vi "Draw Shapes.vi"(0 "Picture in":refnum<vi>, 1 "Commands":cluster{"Time (s)":dbl, T1, "Enabled":bool}[](array[cluster]), 3 "Sample Period (s)":dbl=0.02, 5 "Points":cluster{"x":dbl, "y":dbl, "th":dbl}[](array[cluster]), 7 "Valid Path?":bool=TRUE, 9 "new picture in":picture, 11 "Results":T4, 13 "Output Point":T3, 14 "Path Points":cluster{"x":dbl, "y":dbl}[](array[cluster])) -> (4 "new picture out":picture)   [LabVIEW 2023]
uses:
  Types/Single Cmd Info.ctl
  <vilib>/picture/picture.llb/imagedata.ctl
  Global Settings.vi
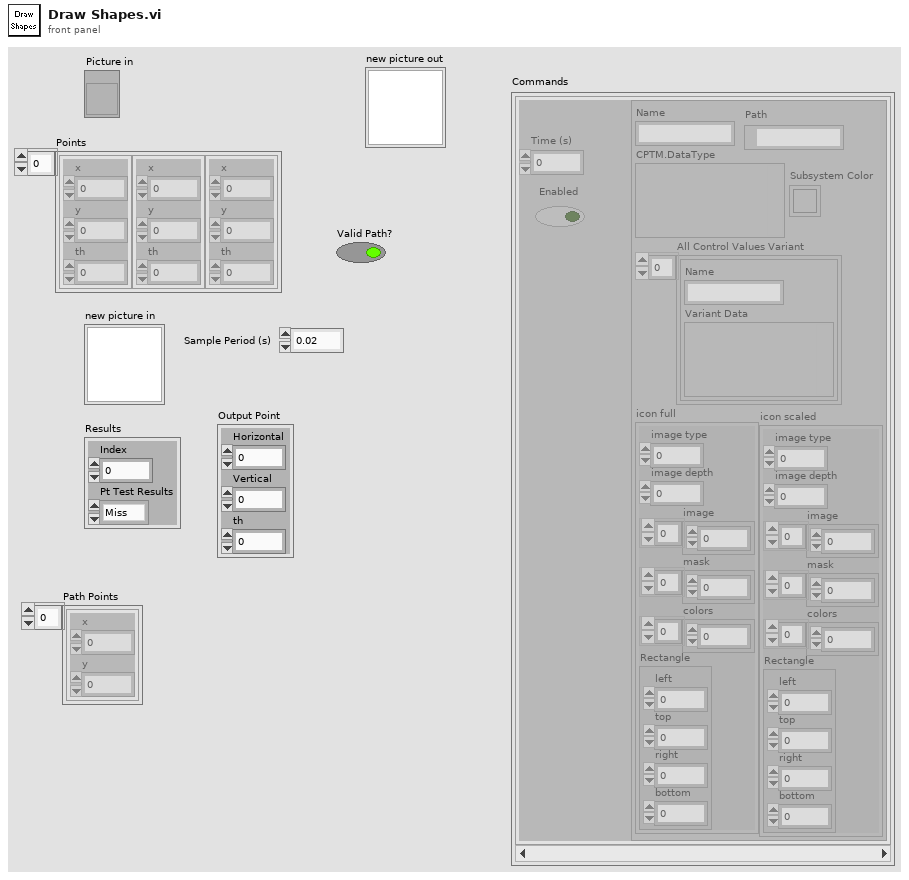
[diagram p1: front panel]
types:
  T1 = typedef "Single Cmd Info.ctl" = cluster{"Name":string, "CPTM.DataType":variant, "All Control Values Variant":cluster{"Name":string, "Variant Data":variant}[], "icon full":T2, "icon scaled":T2, "Path":path, "Subsystem Color":u32}
  T2 = typedef "imagedata.ctl" = cluster{"image type":i32, "image depth":i32, "image":u8[], "mask":u8[], "colors":u32[], "Rectangle":cluster{"left":i16, "top":i16, "right":i16, "bottom":i16}}
  T3 = cluster{"Horizontal":dbl, "Vertical":dbl, "th":dbl}
  T4 = cluster{"Index":i32, "Pt Test Results":enum16{"Miss", "Rect Hit", "Arrow Hit"}}
  T5 = typedef "LVPositionTypeDef.ctl" = cluster{"Left":i32, "Top":i32}
  T6 = typedef "LVBoundsTypeDef.ctl" = cluster{"Width":u32, "Height":u32}
  T7 = cluster{"left":i16, "top":i16, "right":i16, "bottom":i16}
  T8 = cluster{"Horizontal":dbl, "Vertical":dbl, "Horizontal":dbl, "Vertical":dbl}
  T9 = cluster{i32, "Pt Test Results":enum16{"Miss", "Rect Hit", "Arrow Hit"}}
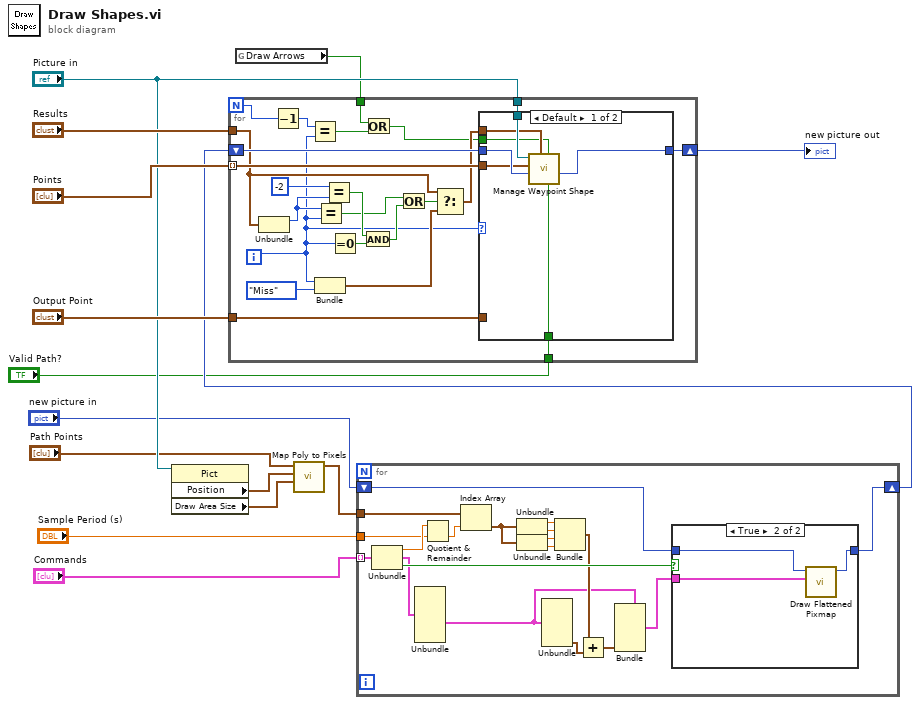
[diagram p0: block diagram]
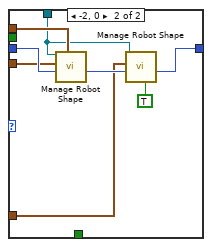
[diagram p3: hidden frame]
diagram:
  n1 = property on="Property Node" class="Pict"(reference="Picture in") -> ("Position"=w9:T5, "Draw Area Size"=w10:T6)  [unwired: 1 in, 2 out]
  n2 = global read "Global Settings.vi" "Draw Arrows"() -> (w2:bool)
  n3 = call "Map Poly to Pixels.vi"("Draw Area Size"=w10, "Position"=w9, "Coords"="Path Points") -> ("Coords"=w7:cluster{"Horizontal":dbl, "Vertical":dbl}[])  [unwired: 8 in]
  n4 = for {
    shift-right: [w27] -> w4
    shift-left: "new picture in" -> [w29]
    tunnel: "Commands" -> [w34] mode=indexing
    tunnel: w7 -> [w33]
    tunnel: "Sample Period (s)" -> [w31]
    n5 = Unbundle(w34) -> ("Time (s)"=w32:dbl, w25:T1, "Enabled"=w28:bool)
    n6 = Unbundle(w25) -> ("icon scaled"=w17:T2)  [unwired: 6 out]
    n7 = Quotient & Remainder(x=w32, y=w31) -> (floor(x/y)=w30:dbl)  [unwired: 1 out]
    n8 = Index Array(array=w33, index=w30) -> (element=w16:cluster{"Horizontal":dbl, "Vertical":dbl})
    n9 = Unbundle(w16) -> ("Horizontal"=w24:dbl, "Vertical"=w23:dbl)
    n10 = Unbundle(w16) -> ("Horizontal"=w22:dbl, "Vertical"=w21:dbl)
    n11 = Unbundle(w17) -> ("Rectangle"=w19:T7)  [unwired: 5 out]
    n12 = Bundle("Horizontal"=w24, "Vertical"=w23, "Horizontal"=w22, "Vertical"=w21) -> (w18:T8)  [unwired: 1 in]
    n13 = Add(x=w18, y=w19) -> (x+y=w26:cluster{dbl, dbl, dbl, dbl})
    n14 = Bundle(cluster=w17, "Rectangle"=w26) -> (w20:T2)  [unwired: 5 in]
    n15 = case shown="True" w28 {
      tunnel: [w35 w36] -> w27
      tunnel: w29 -> [w35 w37]
      tunnel: w20 -> [_ w38]
      frame False {
      }
      frame True {
        n16 = call <vilib>:"Draw Flattened Pixmap.vi"("image data"=w38, "picture"=w37) -> ("new picture"=w36:picture)  [unwired: 7 in]
      }
    }
  }
  n17 = for {
    N -> [w46]
    tunnel: "Points" -> [w61] mode=indexing
    shift-right: [w60] -> w3
    shift-left: w4 -> [w59]
    tunnel: "Picture in" -> [w58]
    tunnel: "Results" -> [w55]
    tunnel: "Output Point" -> [w43]
    tunnel: w2 -> [w40]
    tunnel: "Valid Path?" -> [w39]
    i -> [w44]
    n18 = Unbundle(w55) -> ("Index"=w51:i32)  [unwired: 1 out]
    n19 = Decrement(x=w46) -> (x-1=w45:i32)
    n20 = Equal?(x=w45, y=w44) -> (x = y?=w42:bool)
    n21 = Bundle(w44, "Pt Test Results"=enum16{"Miss", "Rect Hit", "Arrow Hit"}."Miss") -> (w56:T9)  [unwired: 1 in]
    n22 = Equal?(x=w51, y=w44) -> (x = y?=w48:bool)
    n23 = Equal?(x=-2, y=w51) -> (x = y?=w50:bool)
    n24 = Equal To 0?(x=w44) -> (x = 0?=w53:bool)
    n25 = And(x=w50, y=w53) -> (x .and. y?=w49:bool)
    n26 = Or(x=w40, y=w42) -> (x .or. y?=w41:bool)
    n27 = Or(x=w48, y=w49) -> (x .or. y?=w47:bool)
    n28 = Select(t=w55, s=w47, f=w56) -> (s? t:f=w57:T4)
    n29 = case shown="Default" w44 {
      tunnel: w61 -> [w64 w75]
      tunnel: [w67 w72] -> w60
      tunnel: w59 -> [w68 w76]
      tunnel: w58 -> [w66 w70]
      tunnel: w57 -> [w65 w74]
      tunnel: w41 -> [w63 _]
      tunnel: w43 -> [_ w71]
      tunnel: w39 -> [w62 _]
      frame Default {
        n30 = call "Manage Waypoint Shape.vi"("Valid Path?"=w62, "Draw Arrow"=w63, "Drawing Options"=w65, "new picture in"=w68, "Waypoint Position (ft)"=w64, "Pict Ref"=w66) -> ("new picture out"=w67:picture)  [unwired: 4 in, 1 out]
      }
      frame -2, 0 {
        n31 = call "Manage Robot Shape.vi"("Drawing Options"=w74, "new picture in"=w76, "Robot Position (ft)"=w75, "Pict Ref"=w70) -> ("new picture out"=w73:picture)  [unwired: 5 in, 2 out]
        n32 = call "Manage Robot Shape.vi"("Lighter"=TRUE ("Outline"), "new picture in"=w73, "Robot Position (ft)"=w71, "Pict Ref"=w70) -> ("new picture out"=w72:picture)  [unwired: 5 in, 2 out]
      }
    }
  }
  "new picture out" <- w3
